vi "Initialize.vi"(2 "XRef":refnum<vi>) -> (1 "State Out":T1)   [LabVIEW 2012, in "OpenG FilterArray.xnode"]
uses:
  OpenG FilterArray.xnode
  State.ctl
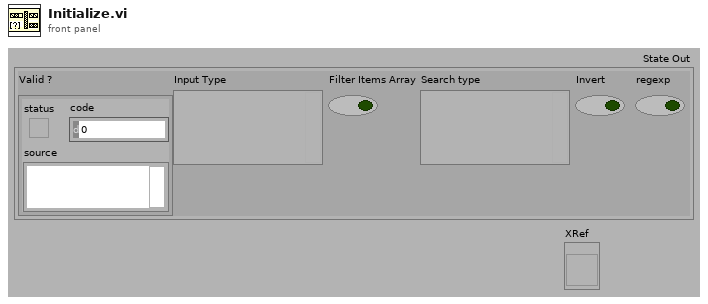
[diagram p1: front panel]
types:
  T1 = typedef "OpenG FilterArray.xnode/State.ctl" = cluster{"Valid ?":errorcluster, "Input Type":variant, "Filter Items Array":bool, "Search type":variant, "Invert":bool, "regexp":bool}
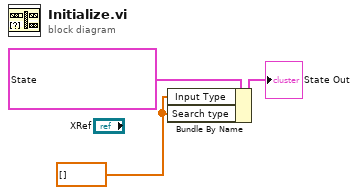
[diagram p0: block diagram]
diagram:
  w1 = dbl[] []
  n1 = Bundle By Name(cluster=T1 {"Valid ?"={"status"=FALSE, "code"=0, "source"="Initialised"}, "Input Type"=variant, "Filter Items Array"=FALSE, "Search type"=variant, "Invert"=FALSE, "regexp"=FALSE} ("State Out"), "Input Type"=w1, "Search type"=w1) -> (→"State Out":T1)
